vi "set Swept SA - Sweep Count.vi"(8 "error in (no error)":errorcluster, 10 "Sweep Count":u32, 11 "FSV-40N in":refnum<class "FSV-40N.lvclass">) -> (0 "error out":errorcluster, 3 "FSV-40N out":refnum<class "FSV-40N.lvclass">)   [LabVIEW 2023, in "Spectrum Analyzer.lvlib" / "FSV-40N.lvclass"]
doc: "This command defines the number of sweeps started with single sweep, which are\nused for calculating the average or maximum value. If the values 0 or 1 are set, one\nsweep is performed.\n\n* For FSV-40\n1) Parameters:\n<NumberSweeps> 0 to 32767\n *RST: 0 (GSM: 200, PHN:1)\nExample: SWE:COUN 64\n Sets the number of sweeps to 64.\n INIT:CONT OFF\n Switches to single sweep mode.\n INIT;*WAI\n Starts a sweep and waits for its end."
uses:
  FSV-40N.lvclass
  FSV-40N.lvclass/FSV-40N.ctl
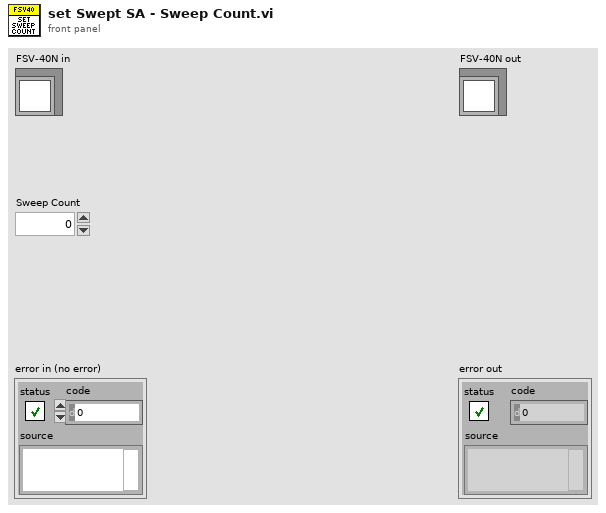
[diagram p1: front panel]
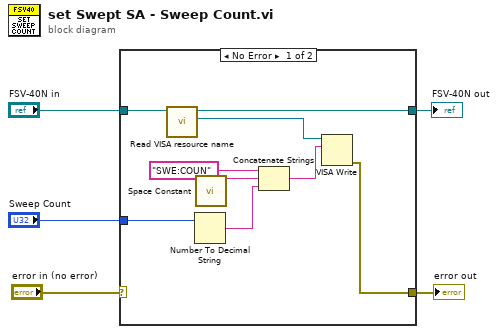
[diagram p0: block diagram]
diagram:
  n1 = case shown="No Error" "error in (no error)" {
    selector: "error in (no error)" -> [_ w15]
    tunnel: "FSV-40N in" -> [w13 w16]
    tunnel: [w7 w16] -> w3
    tunnel: [w6 w15] -> w2
    tunnel: "Sweep Count" -> [w14 _]
    frame No Error {
      n2 = call "Read VISA resource name.vi"("FSV-40N in"=w13) -> ("VISA resource name"=w12:refnum<visa-resource-name>, "FSV-40N out"=w7:refnum<class "FSV-40N.lvclass">)  [unwired: 8 in, 1 out]
      n3 = Number To Decimal String(number=w14) -> (decimal integer string=w9:string)  [unwired: 1 in]
      n4 = call <vilib>:"Space Constant.vi"() -> ("String"=w10:string)
      n5 = Concatenate Strings("SWE:COUN" ("string"), w10, w9) -> (w8:string)
      n6 = VISA Write(VISA resource name=w12, write buffer=w8) -> (error out=w6:errorcluster)  [unwired: 1 in, 2 out]
    }
    frame Error {
    }
  }
  "error out" <- w2
  "FSV-40N out" <- w3
